vi "Own20261012_SetPropertyItemWrite.vi"() -> ()   [LabVIEW 2024]
panel:
  out "error out":errorcluster caption="错误输出"
  in  "is_write":bool
  in  "property_item_id":u32
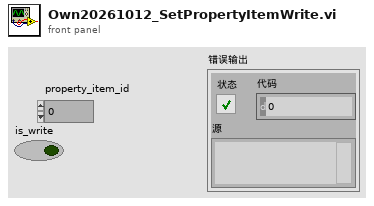
[diagram p1: front panel]
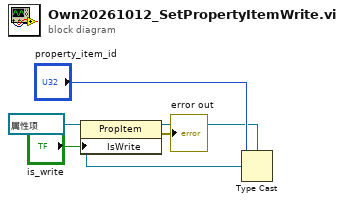
[diagram p0: block diagram]
diagram:
  n1 = Type Cast(type=refnum<vi> refnum ("引用"), x="property_item_id") -> (*(type *) &x=w3:refnum<vi>)
  n2 = property class="PropItem"(reference=w3, "IsWrite"="is_write") -> (error out=→"error out":errorcluster)  [unwired: 1 in, 1 out]
